vi "Script Processing.vi"(4 "init":bool, 6 "buffer size (samples) : Ns":i32=8192 min=1024 step=1024, 7 "VC Handle":T1=-1, 8 "error in":errorcluster, 9 "Sound Rate : rate":enum16{"11025", "22050", "44100"}(ring), 10 "data in":dbl[](array[numeric]), 11 "script":string) -> (0 "error out":errorcluster, 2 "data out":dbl[](array[numeric]), 5 "dup VC Handle":T1=-1)   [LabVIEW 2021]
doc: "The main processing VI writes input variables, executes a script and returns resulting value.\n\n::: CalcExpress Toolkit :::\nCopyright (c) 2000-2026 Konstantin Shifershteyn. All rights reserved."
uses:
  vi.lib/addons/CalcExpress/cetypes.llb/VarMan Variable Context Handle.ctl
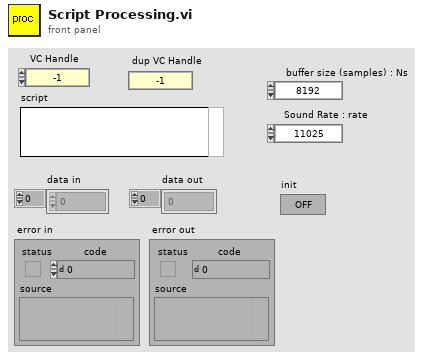
[diagram p1: front panel]
types:
  T1 = typedef "VarMan Variable Context Handle.ctl" = i32
  T2 = enum16{"create", "destroy", "set value", "get value"}
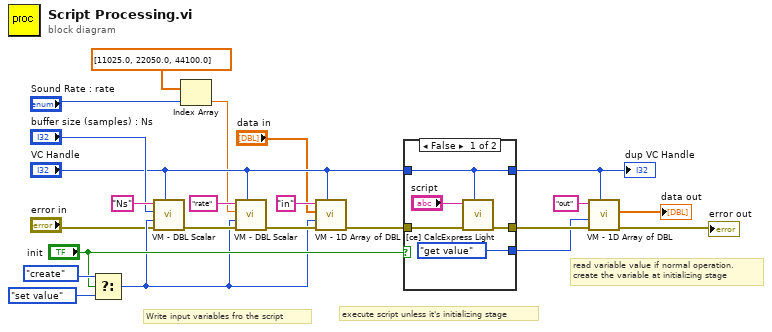
[diagram p0: block diagram]
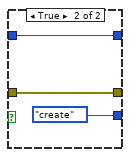
[diagram p2: hidden frame]
diagram:
  # "read variable value if normal operation.\ncreate the variable at initializing stage"
  # "execute script unless it's initializing stage"
  # "Write input variables fro the script"
  n1 = Select(t=T2."create" ("cmd"), s="init", f=T2."set value" ("cmd")) -> (s? t:f=w12:T2)
  n2 = call "VM - DBL Scalar.vi"("VC Handle"="VC Handle", "error in"="error in", "cmd"=w12, "value in"="buffer size (samples) : Ns", "name_spec"="Ns" ("name")) -> ("error out"=w22:errorcluster)  [unwired: 1 in, 5 out]
  n3 = Index Array(array=dbl[] [11025.0, 22050.0, 44100.0], index="Sound Rate : rate") -> (element=w5:dbl)
  n4 = call "VM - DBL Scalar.vi"("VC Handle"="VC Handle", "error in"=w22, "cmd"=w12, "value in"=w5, "name_spec"="rate" ("name")) -> ("error out"=w23:errorcluster)  [unwired: 1 in, 5 out]
  n5 = call "VM - 1D Array of DBL.vi"("VC Handle"="VC Handle", "error in"=w23, "cmd"=w12, "value in"="data in", "name_spec"="in" ("name in")) -> ("error out"=w14:errorcluster)  [unwired: 1 in, 5 out]
  n6 = case shown="False" "init" {
    tunnel: w14 -> [w28 w30]
    tunnel: [w26 w30] -> w11
    tunnel: "VC Handle" -> [w24 w31]
    tunnel: [w24 w31] -> w8
    tunnel: [T2."get value" ("cmd") T2."create" ("cmd")] -> w10
    frame False {
      n7 = call "[ce] CalcExpress Light.vi"("VC Handle"=w24, "error in"=w28, "expression"="script") -> ("error out"=w26:errorcluster)  [unwired: 6 in, 2 out]
    }
    frame True {
    }
  }
  "dup VC Handle" <- w8
  n8 = call "VM - 1D Array of DBL.vi"("VC Handle"=w8, "error in"=w11, "cmd"=w10, "name_spec"="out" ("name in")) -> ("error out"=→"error out":errorcluster, "value out"=→"data out":dbl[])  [unwired: 2 in, 4 out]
